vi "UDP Write.vi"(5 "对方端口":u16=12345, 7 "地址":u32, 8 "错误输入（无错误）":errorcluster, 10 "数据输入":string, 11 "连接ID":refnum<k16>) -> (0 "错误输出":errorcluster, 3 "连接ID输出":refnum<k16>)   [LabVIEW 2026, in "UI-距离测量.lvlib" / "UDP.lvlib"]
uses:
  UDP.lvlib
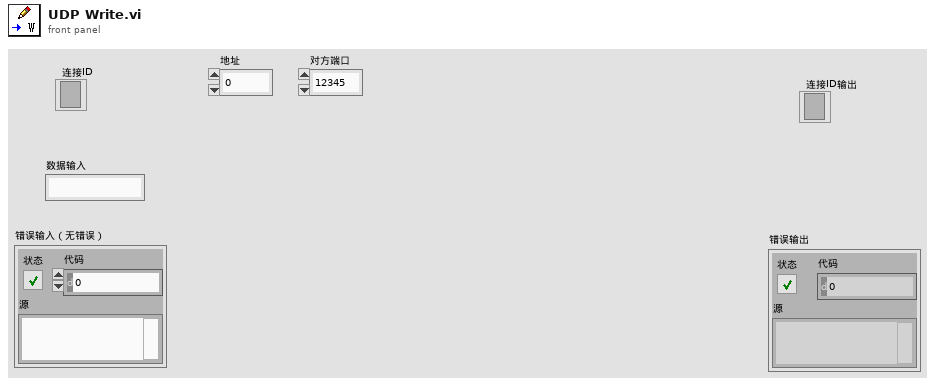
[diagram p1: front panel]
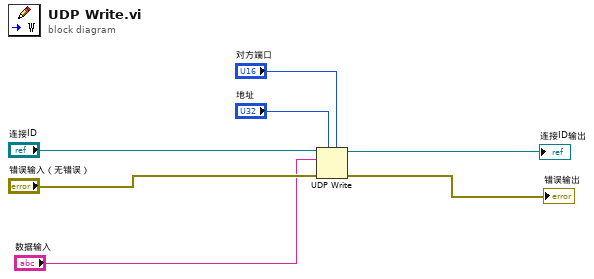
[diagram p0: block diagram]
diagram:
  n1 = UDP Write(address="地址", port or service name="对方端口", connection ID="连接ID", data in="数据输入", 8:"错误输入（无错误）") -> (error out=→"错误输出":errorcluster, 3:→"连接ID输出":refnum<k16>)  [unwired: 1 in]
